vi "UE_Clamp_To_Limits.vi"(3 "maximum":dbl, 4 "minimum":dbl, 5 "value":dbl) -> (1 "original_in_range":bool, 2 "clamped":dbl)   [LabVIEW 2026]
doc: "INTENT: Coerce numeric target into validated bounds and report whether original target was inside. INPUTS: value (double), minimum (double), maximum (double). OUTPUTS: clamped (double), original_in_range (bool). DESIGN CONSTRAINT: Clamping a setpoint does not grant permission to issue a hardware command. REQUIREMENTS: SRS-F-021. No physical hardware side effects. Acceptance requires native LabVIEW compilation and behavioral testing."
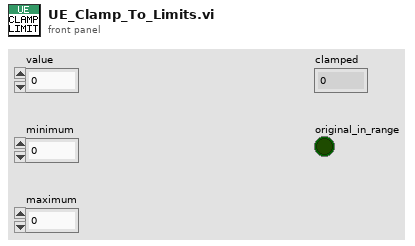
[diagram p1: front panel]
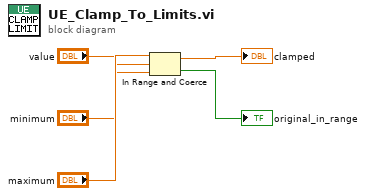
[diagram p0: block diagram]
diagram:
  n1 = In Range and Coerce(upper limit="maximum", x="value", lower limit="minimum") -> (coerced(x)=→"clamped":dbl, In Range?=→"original_in_range":bool)
